vi "Read status.vi"(8 "error in (no error)":errorcluster, 11 "Mechanism in":refnum<class "Mechanism.lvclass">) -> (0 "error out":errorcluster, 2 "status":T1, 3 "Mechanism out":refnum<class "Mechanism.lvclass">)   [LabVIEW 2018, in "Mechanism.lvclass"]
uses:
  Mechanism.lvclass
  Mechanism.lvclass/Mechanism.ctl
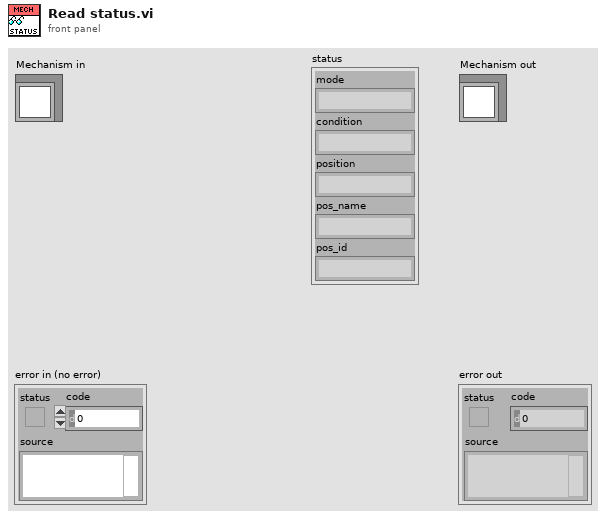
[diagram p1: front panel]
types:
  T1 = cluster{"mode":string, "condition":string, "position":string, "pos_name":string, "pos_id":string}
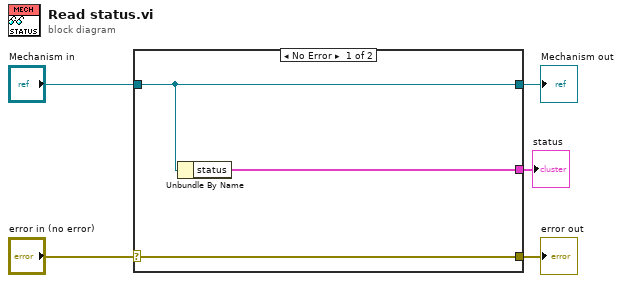
[diagram p0: block diagram]
diagram:
  n1 = case shown="No Error" "error in (no error)" {
    selector: "error in (no error)" -> [w8 w9]
    tunnel: [w8 w9] -> w4
    tunnel: [w7 w10] -> w2
    tunnel: "Mechanism in" -> [w7 w10]
    tunnel: [w6 _] -> w1
    frame No Error {
      n2 = Unbundle By Name(w7) -> ("status"=w6:T1)
    }
    frame Error {
    }
  }
  "error out" <- w4
  "Mechanism out" <- w2
  "status" <- w1
